vi "pid.vi"() -> ()   [LabVIEW 2015]
uses:
  <vilib>/Instr/_visa.llb/Select Event Type.ctl
  <vilib>/Instr/_visa.llb/VISA Configure Serial Port (Instr).vi
panel:
  out "Waveform Chart":dynamicdata(graph)
  in  "stop":bool
  out "read buffer":string
  in  "Puerto":refnum<visa-resource-name>
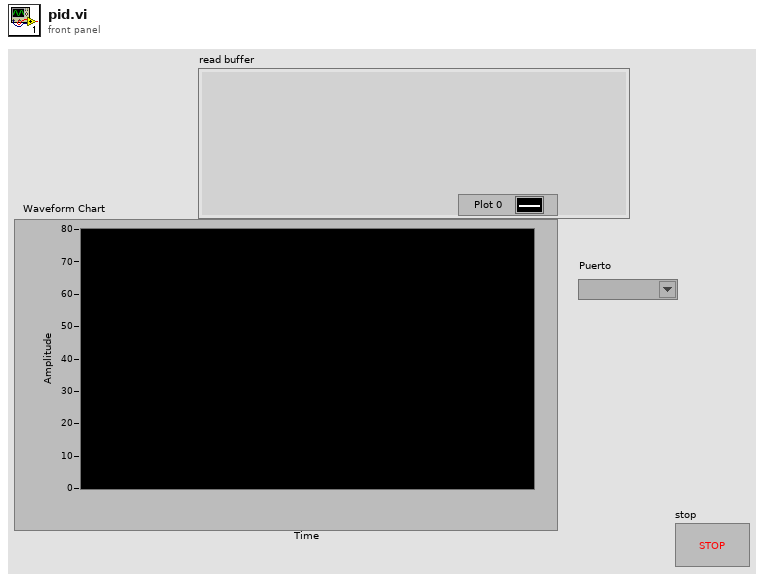
[diagram p1: front panel]
types:
  T1 = typedef "Select Event Type.ctl" = u32
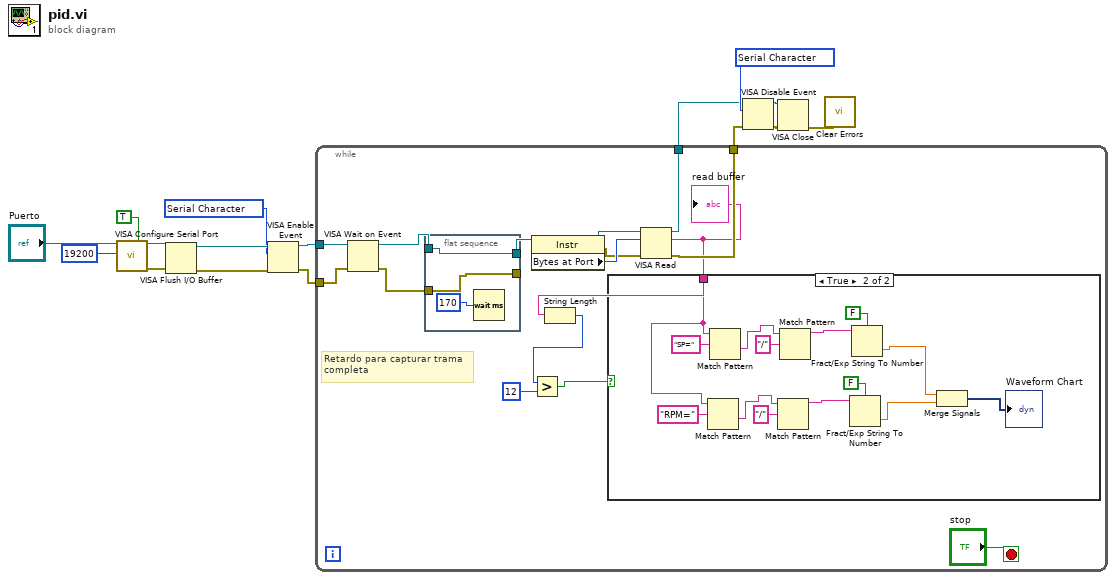
[diagram p0: block diagram]
diagram:
  w4 = T1 1073684533 items=["Service Request"=1073684491, "Trigger"=3221168138, "Clear"=1073684493, "VXI Signal"=1073684512, "VXI/VME Interrupt"=3221168161, "VXI/VME Sysfail"=1073684509, "VXI/VME Sysreset"=1073684510, "GPIB CIC"=1073684498, "GPIB Talk"=1073684499, "GPIB Listen"=1073684500, "PXI Interrupt"=1073684514, "Serial Break"=1073684515, "Serial TermChar"=1073684516, "Serial CTS"=1073684521, "Serial DSR"=1073684522, "Serial DCD"=1073684524, "Serial RI"=1073684526, "Serial Character"=1073684533, "USB Interrupt"=1073684535, "All Enabled"=1073709055] ("Event Type")
  w9 = T1 1073684533 items=["Service Request"=1073684491, "Trigger"=3221168138, "Clear"=1073684493, "VXI Signal"=1073684512, "VXI/VME Interrupt"=3221168161, "VXI/VME Sysfail"=1073684509, "VXI/VME Sysreset"=1073684510, "GPIB CIC"=1073684498, "GPIB Talk"=1073684499, "GPIB Listen"=1073684500, "PXI Interrupt"=1073684514, "Serial Break"=1073684515, "Serial TermChar"=1073684516, "Serial CTS"=1073684521, "Serial DSR"=1073684522, "Serial DCD"=1073684524, "Serial RI"=1073684526, "Serial Character"=1073684533, "USB Interrupt"=1073684535, "All Enabled"=1073709055] ("Event Type")
  n1 = call-poly "VISA Configure Serial Port"("VISA resource name"="Puerto", "Enable Termination\nChar (T)"=TRUE ("Enable Termination\nChar (T)"), "baud rate (9600)"=u32 19200) -> ("VISA resource name out"=w12:refnum<visa-resource-name>, "error out"=w13:errorcluster)  [unwired: 11 in]
  n2 = VISA Flush I/O Buffer(VISA resource name=w12, error in (no error)=w13) -> (VISA resource name out=w11:refnum<visa-resource-name>, error out=w10:errorcluster)  [unwired: 1 in]
  n3 = VISA Enable Event ("VISA Enable \nEvent")(8:w10, 10:w9, 11:w11) -> (0:w7:errorcluster, 3:w8:refnum<visa-resource-name>)  [unwired: 1 out]
  n4 = while {
    tunnel: w8 -> [w25]
    tunnel: w7 -> [w24]
    tunnel: [w23] -> w2
    tunnel: [w22] -> w1
    stop <- "stop" stop-if-true
    # "Retardo para capturar trama\ncompleta"
    n5 = VISA Wait on Event(8:w24, 11:w25) -> (0:w31:errorcluster, 3:w30:refnum<visa-resource-name>)  [unwired: 2 in, 3 out]
    n6 = flat-sequence {
      tunnel: w30 -> [w48]
      tunnel: [w48] -> w27
      tunnel: [w47] -> _
      tunnel: w31 -> [w47]
      frame #0 {
        n7 = Wait (ms)(milliseconds to wait=u32 170) -> ()  [unwired: 1 out]
      }
    }
    n8 = property class="Instr"(reference=w27) -> (reference out=w29:refnum<visa-resource-name>, error out=w26:errorcluster, "Bytes at Port"=w28:u32)  [unwired: 1 in]
    n9 = VISA Read(VISA resource name=w29, byte count=w28, error in (no error)=w26) -> (VISA resource name out=w23:refnum<visa-resource-name>, read buffer=w20:string, error out=w22:errorcluster)  [unwired: 1 out]
    "read buffer" <- w20
    n10 = String Length(string=w20) -> (length=w19:i32)
    n11 = Greater?(x=w19, y=12) -> (0:w17:bool)
    n12 = case shown="True" w17 {
      tunnel: w20 -> [_ w32]
      frame False {
      }
      frame True {
        n13 = Match Pattern(string=w32, regular expression="RPM=") -> (after substring=w39:string)  [unwired: 1 in, 3 out]
        n14 = Match Pattern(string=w32, regular expression="SP=") -> (after substring=w42:string)  [unwired: 1 in, 3 out]
        n15 = Match Pattern(string=w39, regular expression="/") -> (before substring=w40:string)  [unwired: 1 in, 3 out]
        n16 = Match Pattern(string=w42, regular expression="/") -> (before substring=w41:string)  [unwired: 1 in, 3 out]
        n17 = Fract/Exp String To Number(use system decimal point (T)=FALSE, string=w40) -> (number=w34:dbl)  [unwired: 2 in, 1 out]
        n18 = Fract/Exp String To Number(use system decimal point (T)=FALSE, string=w41) -> (number=w35:dbl)  [unwired: 2 in, 1 out]
        n19 = Merge Signals(w35, w34) -> (→"Waveform Chart":dynamicdata)
      }
    }
  }
  n20 = VISA Disable Event ("VISA Disable \nEvent")(8:w1, 10:w4, 11:w2) -> (0:w6:errorcluster, 3:w5:refnum<visa-resource-name>)  [unwired: 1 out]
  n21 = VISA Close(VISA resource name=w5, error in (no error)=w6) -> (error out=w3:errorcluster)
  n22 = call <vilib>:"Clear Errors.vi"("error in (no error)"=w3) -> ()  [unwired: 5 in, 2 out]
